vi "FX_BuildFrame.vi"(10 "Content":string, 11 "Command":string) -> (3 "Frame":string)   [LabVIEW 2018]
doc: "Use this template to build a VI to use as a subVI."
panel:
  # "說明：組編程協定封包：STX + 命令 + 內容 + ETX + 和\n校驗。和校驗＝STX 之後到 ETX 的總和取低 8 位。"
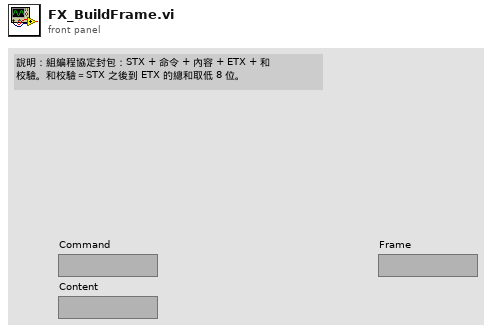
[diagram p1: front panel]
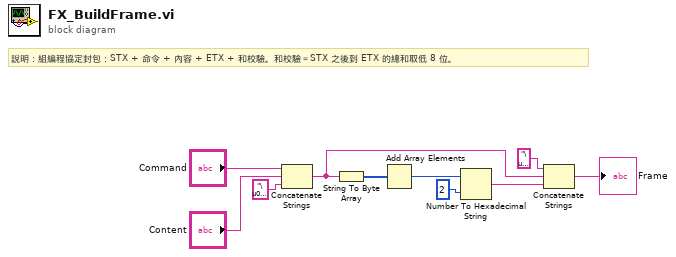
[diagram p0: block diagram]
diagram:
  # "說明：組編程協定封包：STX + 命令 + 內容 + ETX + 和校驗。和校驗＝STX 之後到 ETX 的總和取低 8 位。"
  n1 = Concatenate Strings("Command", "Content", "\u0003") -> (w7:string)
  n2 = String To Byte Array(string=w7) -> (unsigned byte array=w6:u8[])
  n3 = Add Array Elements(numeric array=w6) -> (sum=w5:u8)
  n4 = Number To Hexadecimal String(1:i16 2 ("width (-)"), 2:w5) -> (0:w2:string)
  n5 = Concatenate Strings("\u0002", w7, w2) -> (→"Frame":string)
